vi "Test_API_Open_Close.vi"() -> ()   [LabVIEW 2021]
doc: "A3 test: Init ? Frames_Create ? Open ? Status ? hold ? Close ? Status, through the API only."
uses:
  api/CANsub_Channel/CANsub_Channel.lvclass
  common/Typedefs/CANsub_connection.ctl
  common/CANsub_Common.lvlib
  common/Typedefs/CANsub_Bit_Rates.ctl
  api/Typedefs/CANsub_Filter.ctl
  api/CANsub_API.lvlib
  api/Typedefs/CANsub_Read_Mode.ctl
  api/Typedefs/CANsub_Ownership.ctl
  api/Typedefs/CANsub_Config.ctl
  api/Typedefs/CANsub_State.ctl
  common/Typedefs/Bit_Timing.ctl
  api/Typedefs/CANsub_Status.ctl
panel:
  out "error out":errorcluster
  out "status closed":T1
  out "status open":T1
  out "frames capacity":i32
  in  "capacity":i32=1756
  in  "hold open (msec)":u32=5000
  in  "config":T4={"connection"={"host"="192.168.0.49", "channel"=2, "cert path"=path "/home/lvuser/cansub_root_cert.crt"}, "bit rates"={"nominal bit rate"=500000, "nominal sample point"=80.0, "data bit rate"=2000000, "data sample point"=80.0}, "listen only"=FALSE, "filters"=[], "read mode"=enum."Poll", "max bytes per read"=4096, "reader FIFO depth"=0, "reader priority"=0, "ownership"=enum."Direct"} {"filters"."f2" format="%.0x"; "filters"."f1" format="%.0x"}
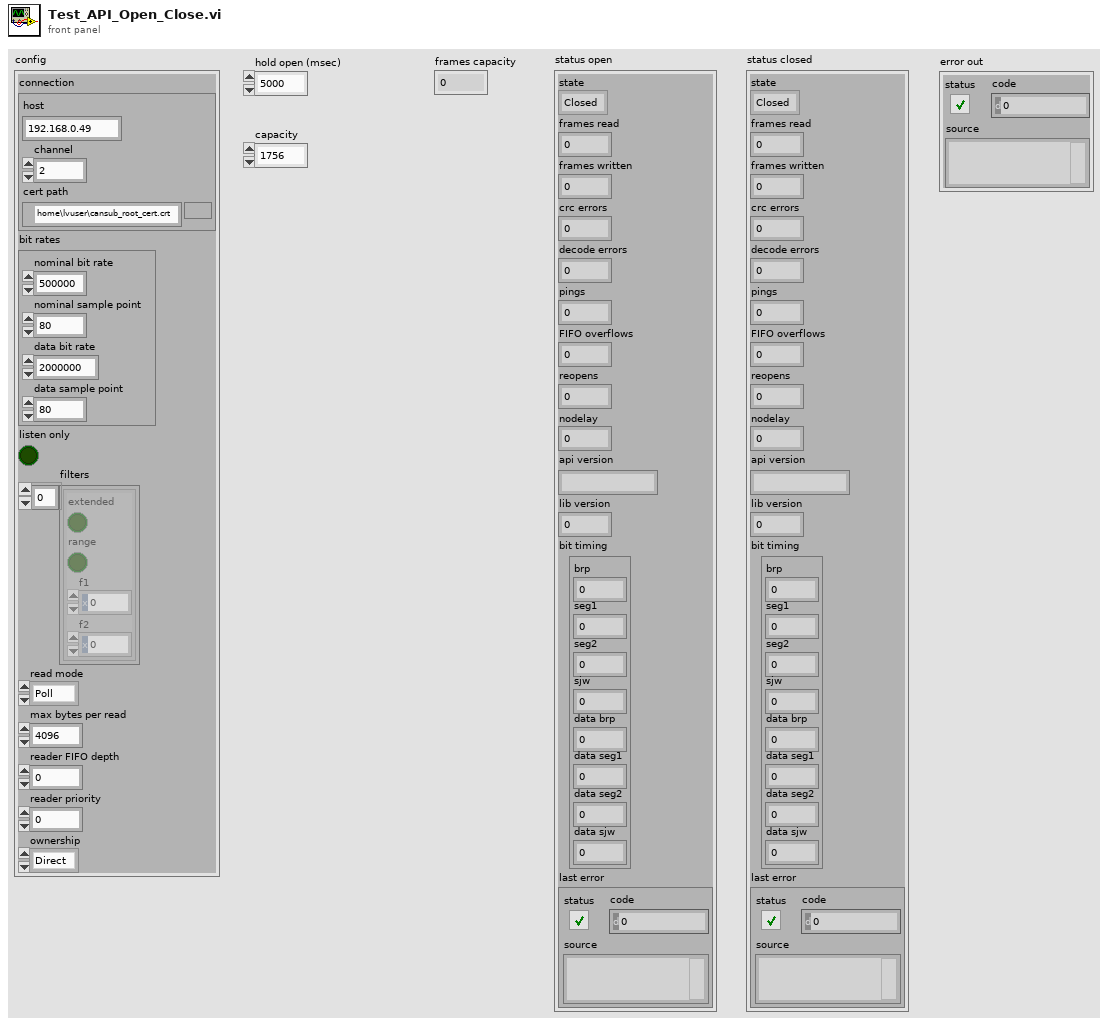
[diagram p1: front panel]
types:
  T1 = typedef "CANsub_API.lvlib/CANsub_Status.ctl" = cluster{"state":T2, "frames read":u32, "frames written":u32, "crc errors":u32, "decode errors":i32, "pings":u32, "FIFO overflows":u32, "reopens":u32, "nodelay":i32, "api version":string, "lib version":u32, "bit timing":T3, "last error":errorcluster}
  T2 = typedef "CANsub_API.lvlib/CANsub_State.ctl" = enum16{"Closed", "Open", "Lost"}
  T3 = typedef "CANsub_Common.lvlib/Bit_Timing.ctl" = cluster{"brp":u16, "seg1":u16, "seg2":u16, "sjw":u16, "data brp":u16, "data seg1":u16, "data seg2":u16, "data sjw":u16}
  T4 = typedef "CANsub_API.lvlib/CANsub_Config.ctl" = cluster{"connection":T5, "bit rates":T6, "listen only":bool, "filters":T7[], "read mode":T8, "max bytes per read":i32, "reader FIFO depth":i32, "reader priority":i32, "ownership":T9}
  T5 = typedef "CANsub_Common.lvlib/CANsub_connection.ctl" = cluster{"host":string, "channel":u8, "cert path":path}
  T6 = typedef "CANsub_Common.lvlib/CANsub_Bit_Rates.ctl" = cluster{"nominal bit rate":u32, "nominal sample point":dbl, "data bit rate":u32, "data sample point":dbl}
  T7 = typedef "CANsub_API.lvlib/CANsub_Filter.ctl" = cluster{"extended":bool, "range":bool, "f1":u32, "f2":u32}
  T8 = typedef "CANsub_API.lvlib/CANsub_Read_Mode.ctl" = enum16{"Poll", "Reader"}
  T9 = typedef "CANsub_API.lvlib/CANsub_Ownership.ctl" = enum16{"Direct", "Shared"}
  T10 = typedef "CANsub_API.lvlib/CANsub_Frames.ctl" = cluster{"count":i32, "t_dev":dbl[], "id":u32[], "flags":u16[], "dlc":u8[], "data len":u8[], "data":u8[]}
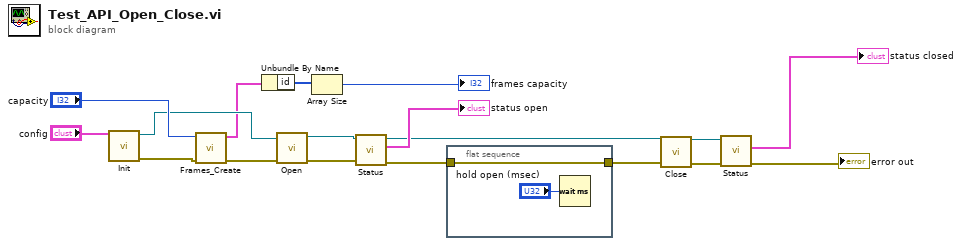
[diagram p0: block diagram]
diagram:
  n1 = call "Init.vi"("config"="config") -> ("error out"=w11:errorcluster, "channel out"=w17:refnum<class "CANsub_Channel.lvclass">)  [unwired: 8 in, 1 out]
  n2 = call "Frames_Create.vi"("error in (no error)"=w11, "capacity"="capacity") -> ("error out"=w10:errorcluster, "frames"=w16:T10)  [unwired: 8 in]
  n3 = Unbundle By Name(w16) -> ("id"=w15:u32[])
  n4 = call-dynamic "Open.vi"("error in (no error)"=w10, "channel in"=w17) -> ("error out"=w9:errorcluster, "channel out"=w13:refnum<class "CANsub_Channel.lvclass">)  [unwired: 8 in]
  n5 = Array Size(array=w15) -> (size(s)=→"frames capacity":i32)
  n6 = call-dynamic "Status.vi"("error in (no error)"=w9, "channel in"=w13) -> ("error out"=w7:errorcluster, "status"=→"status open":T1, "channel out"=w3:refnum<class "CANsub_Channel.lvclass">)  [unwired: 7 in]
  n7 = flat-sequence {
    tunnel: [w19] -> w8
    tunnel: w7 -> [w19]
    frame #0 {
      n8 = Wait (ms)(milliseconds to wait="hold open (msec)") -> ()  [unwired: 1 out]
    }
  }
  n9 = call-dynamic "Close.vi"("error in (no error)"=w8, "channel in"=w3) -> ("error out"=w5:errorcluster, "channel out"=w4:refnum<class "CANsub_Channel.lvclass">)  [unwired: 8 in]
  n10 = call-dynamic "Status.vi"("error in (no error)"=w5, "channel in"=w4) -> ("error out"=→"error out":errorcluster, "status"=→"status closed":T1)  [unwired: 7 in, 1 out]
